vi "CreatePathWriteTrajCSVFile_Example.vi"(11 "Max Velocity M/S":dbl=3.2 format="%17.3f") -> (1 "PathPlannerTrajectory":T2 {"States"."TargetHolonomicRotation"."SIN" format="%13.4f"; "States"."TargetHolonomicRotation"."COS" format="%13.4f"; "States"."TargetHolonomicRotation"."VALUE" format="%13.4f"; "States"."Heading"."SIN" format="%13.4f"; "States"."Heading"."COS" format="%13.4f"; "States"."Heading"."VALUE" format="%13.4f"; "States"."PositionMeters"."Y" format="%14.3f"; "States"."PositionMeters"."X" format="%14.3f"}, 2 "Trajectory State\nCount":i32, 3 "TotalTImeSecs":dbl)   [LabVIEW 2019]
uses:
  <vilib>/Rock Robotics/WPI/ThirdParty/JAS_Junk/TrajLib/Trajectory_Library.lvlib
  <vilib>/Rock Robotics/WPI/ThirdParty/MJansen/PathPlanner/PathPlanner24.lvlib
  <vilib>/Rock Robotics/WPI/ThirdParty/JAS_Junk/TrajLib/TypeDef/TRANSLATION2D.ctl
  <vilib>/Rock Robotics/WPI/ThirdParty/JAS_Junk/TrajLib/TypeDef/ROTATION2D.ctl
  <vilib>/Rock Robotics/WPI/ThirdParty/MJansen/PathPlanner/TypeDef/PathPlannerPathConstraints.ctl
  <vilib>/Rock Robotics/WPI/ThirdParty/MJansen/PathPlanner/TypeDef/PathPlannerTrajectoryState.ctl
  <vilib>/Rock Robotics/WPI/ThirdParty/MJansen/PathPlanner/TypeDef/PathPlannerTrajectory.ctl
panel:
  in  "Trajectory CSV File Name":path=path "sample.csv"
  in  "Optional Comment":string="Sample PathPlanner Trajectory"
  in  "Write File":bool
  out "Trajectory\nWrite error":errorcluster
  in  "End Angle Degrees":dbl format="%#_13g"
  in  "End Velocity M/S":dbl format="%#_13g"
  in  "Start Angual Vel Rad/S":dbl format="%#_13g"
  in  "Start Y Vel M/S":dbl format="%#_13g"
  in  "Start X Vel M/S":dbl format="%#_13g"
  in  "MaxAngularAccel Radians.Sec^2":dbl=2.4 format="%17.3f"
  in  "Point 4":T1={"X Meters"=3.0, "Y Meters"=3.0, "Heading  Deg"=90.0} {"Heading  Deg" format="%13.3f"; "Y Meters" format="%13.3f"; "X Meters" format="%13.3f"}
  in  "Point 3":T1={"X Meters"=3.0, "Y Meters"=2.7, "Heading  Deg"=90.0} {"Heading  Deg" format="%13.3f"; "Y Meters" format="%13.3f"; "X Meters" format="%13.3f"}
  in  "Point 2":T1={"X Meters"=1.3, "Y Meters"=1.0, "Heading  Deg"=0.0} {"Heading  Deg" format="%13.3f"; "Y Meters" format="%13.3f"; "X Meters" format="%13.3f"}
  out "Path\nCreation\nError":bool
  out "Trajectory":cluster{dbl[], dbl[]}(graph)
  in  "Initial Point":T1={"X Meters"=1.0, "Y Meters"=1.0, "Heading  Deg"=0.0} {"Heading  Deg" format="%13.3f"; "Y Meters" format="%13.3f"; "X Meters" format="%13.3f"}
  in  "MaxAcceleration M/S^2":dbl=2.8 format="%17.1f"
  in  "MaxAngularVel  Radians/Sec":dbl=1.8 format="%17.3f"
  # "Create PathPlanner Path/Trajectory Sample"
  # "This VI is designed to be called by BEGIN.VI, but can be executed directly to test trajectory parameters."
  # "CREATED TRAJECTORY INFORMATION"
  # "PATH CONFIGURATION"
  # "PATH DEFINITION"
  # "WRITE TRAJECTORY TO FILE"
  # "There can be as many points as needed."
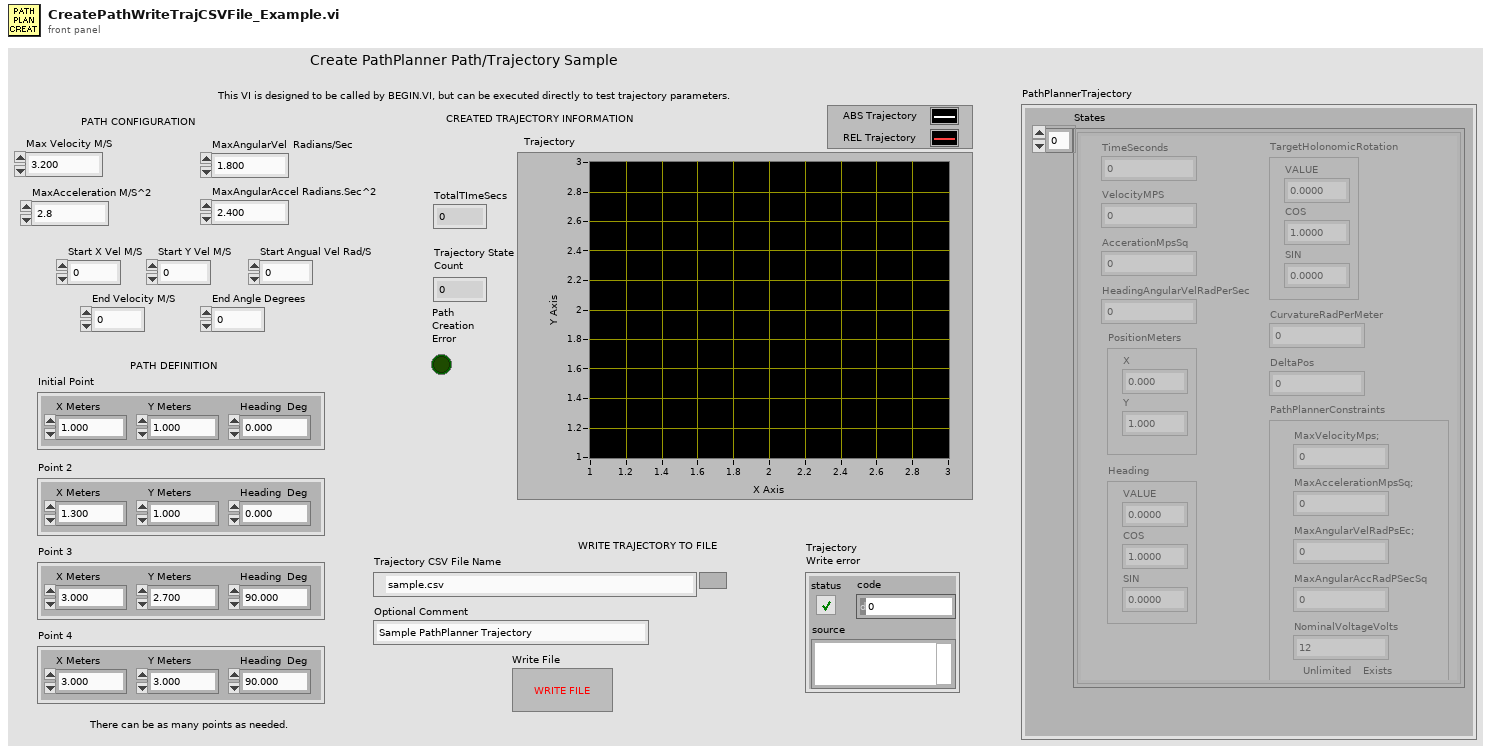
[diagram p1: front panel]
types:
  T1 = cluster{"X Meters":dbl, "Y Meters":dbl, "Heading  Deg":dbl}
  T2 = typedef "PathPlanner24.lvlib/PathPlannerTrajectory.ctl" = cluster{"States":T3[]}
  T3 = typedef "PathPlanner24.lvlib/PathPlannerTrajectoryState.ctl" = cluster{"TimeSeconds":dbl, "VelocityMPS":dbl, "AccerationMpsSq":dbl, "HeadingAngularVelRadPerSec":dbl, "PositionMeters":T4, "Heading":T5, "TargetHolonomicRotation":T5, "CurvatureRadPerMeter":dbl, "PathPlannerConstraints":T6, "DeltaPos":dbl}
  T4 = typedef "Trajectory_Library.lvlib/TRANSLATION2D.ctl" = cluster{"X":dbl, "Y":dbl}
  T5 = typedef "Trajectory_Library.lvlib/ROTATION2D.ctl" = cluster{"VALUE":dbl, "COS":dbl, "SIN":dbl}
  T6 = typedef "PathPlanner24.lvlib/PathPlannerPathConstraints.ctl" = cluster{"MaxVelocityMps;":dbl, "MaxAccelerationMpsSq;":dbl, "MaxAngularVelRadPsEc;":dbl, "MaxAngularAccRadPSecSq":dbl, "Exists":bool, "Unlimited":bool, "NominalVoltageVolts":dbl}
  T7 = typedef "Trajectory_Library.lvlib/POSE2D.ctl" = cluster{"TRANSLATION":T4, "ROTATION":T5}
  T8 = typedef "Trajectory_Library.lvlib/CHASSIS_SPEEDS.ctl" = cluster{"vX":dbl, "vY":dbl, "vOmega":dbl}
  T9 = typedef "PathPlanner24.lvlib/PathPlannerGoalEndState.ctl" = cluster{"VelocityMPS":dbl, "Rotation":T5}
  T10 = typedef "PathPlanner24.lvlib/PathPlannerWaypoint.ctl" = cluster{"prevControl":T4, "anchor":T4, "nextControl":T4, "PrevExists":bool, "NextExists":bool}
  T11 = typedef "PathPlanner24.lvlib/PathPlannerPath.ctl" = cluster{"Reversed":bool, "RotationTargets":T12[], "ConstraintZones":T13[], "EventMarkers":T14[], "GlobalConstraints":T6, "GoalEndState":T9, "AllPoints":T17[], "Name":string, "Waypoints":T10[], "PointTowardsZones":T18[], "IdealStartingState":T19, "IsChoreoPath":bool, "PreventFlipping":bool}
  T12 = typedef "PathPlanner24.lvlib/PathPlannerRotationTarget.ctl" = cluster{"position":dbl, "rotation":T5, "Exists":bool}
  T13 = typedef "PathPlanner24.lvlib/PathPlannerConstraintsZone.ctl" = cluster{"minPosition":dbl, "maxPosition":dbl, "Constraints":T6, "Present":bool}
  T14 = typedef "PathPlanner24.lvlib/PathPlannerEventMarker.ctl" = cluster{"Position":dbl, "Command":T15, "TriggerName":string, "EndPosition":dbl}
  T15 = typedef "PathPlanner24.lvlib/PathPlannerCommandUtil.ctl" = cluster{"waitTime":dbl, "name":string, "pathName":string, "commands":cluster{"type":T16, "waitTime":dbl, "name":string, "pathName":string}[], "type":T16}
  T16 = typedef "PathPlanner24.lvlib/PathPlanner_CommandUtilType_ENUM.ctl" = enum16{"Unknown", "Wait", "Named", "Path", "Sequential", "Parallel", "Race", "Deadline"}
  T17 = typedef "PathPlanner24.lvlib/PathPlannerPathPoint.ctl" = cluster{"Position":T4, "DistAlongPath":dbl, "MaxV":dbl, "Constraints":T6, "RotationTarget":T12, "WaypointRelativePos":dbl}
  T18 = typedef "PathPlanner24.lvlib/PathPlannerPointTowardsZone.ctl" = cluster{"RotationOffset":T5, "Name":string, "TargetPosition":T4, "MinPosition":dbl, "MaxPosition":dbl}
  T19 = typedef "PathPlanner24.lvlib/PathPlannerIdealStartingState.ctl" = cluster{"VelocityMPS":dbl, "Rotation":T5}
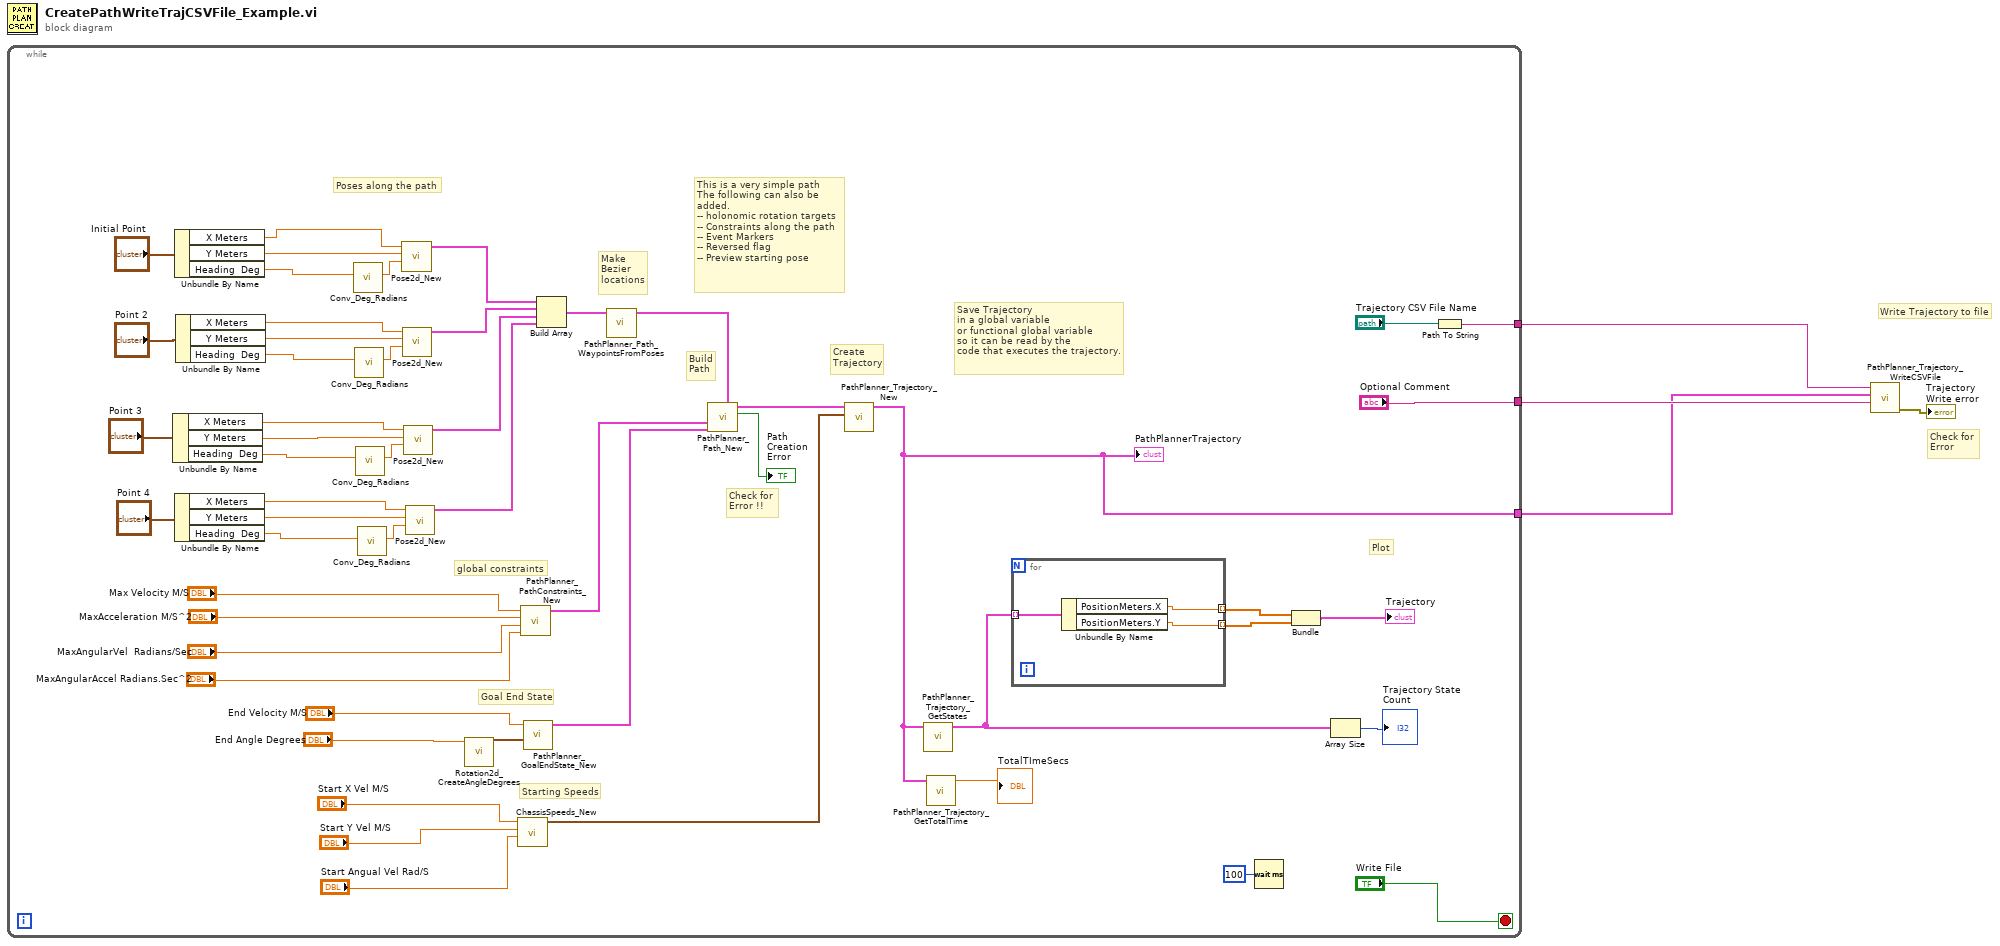
[diagram p0: block diagram]
diagram:
  # "Write Trajectory to file"
  # "Check for\nError"
  n1 = while {
    tunnel: ["Optional Comment"] -> w3
    tunnel: [w8] -> w2
    tunnel: [w7] -> w1
    stop <- "Write File" stop-if-true
    # "This is a very simple path\nThe following can also be\nadded.\n-- holonomic rotation targets\n-- Constraints along the path\n-- Event Markers\n-- Reversed flag\n-- Preview starting pose"
    # "Plot"
    # "Save Trajectory\nin a global variable\nor functional global variable\nso it can be read by the \ncode that executes the trajectory."
    # "Create\nTrajectory"
    # "Check for\nError !!"
    # "Starting Speeds"
    # "Goal End State"
    # "global constraints"
    # "Make\nBezier\nlocations"
    # "Build\nPath"
    # "Poses along the path"
    n2 = Unbundle By Name("Point 3") -> ("X Meters"=w21:dbl, "Y Meters"=w20:dbl, "Heading  Deg"=w19:dbl)
    n3 = Unbundle By Name("Initial Point") -> ("X Meters"=w29:dbl, "Y Meters"=w28:dbl, "Heading  Deg"=w27:dbl)
    n4 = Unbundle By Name("Point 4") -> ("X Meters"=w18:dbl, "Y Meters"=w17:dbl, "Heading  Deg"=w16:dbl)
    n5 = Unbundle By Name("Point 2") -> ("X Meters"=w26:dbl, "Y Meters"=w25:dbl, "Heading  Deg"=w24:dbl)
    n6 = call <vilib>:"Conv_Deg_Radians.vi"("Degress"=w27) -> ("Radians"=w38:dbl)  [unwired: 10 in]
    n7 = call <vilib>:"Conv_Deg_Radians.vi"("Degress"=w24) -> ("Radians"=w39:dbl)  [unwired: 10 in]
    n8 = call <vilib>:"Conv_Deg_Radians.vi"("Degress"=w19) -> ("Radians"=w40:dbl)  [unwired: 10 in]
    n9 = call <vilib>:"Conv_Deg_Radians.vi"("Degress"=w16) -> ("Radians"=w41:dbl)  [unwired: 10 in]
    n10 = call <vilib>:"Pose2d_New.vi"("Heading"=w38, "Y"=w28, "X"=w29) -> ("out POSe"=w42:T7)  [unwired: 8 in]
    n11 = call <vilib>:"Pose2d_New.vi"("Heading"=w39, "Y"=w25, "X"=w26) -> ("out POSe"=w43:T7)  [unwired: 8 in]
    n12 = call <vilib>:"Pose2d_New.vi"("Heading"=w40, "Y"=w20, "X"=w21) -> ("out POSe"=w44:T7)  [unwired: 8 in]
    n13 = call <vilib>:"Pose2d_New.vi"("Heading"=w41, "Y"=w17, "X"=w18) -> ("out POSe"=w45:T7)  [unwired: 8 in]
    n14 = call <vilib>:"Rotation2d_CreateAngleDegrees.vi"("Angle_Degrees"="End Angle Degrees") -> ("ROTATION"=w49:T5)  [unwired: 10 in]
    n15 = call <vilib>:"ChassisSpeeds_New.vi"("vAngular"="Start Angual Vel Rad/S", "vY"="Start Y Vel M/S", "vX"="Start X Vel M/S") -> ("CHASSIS"=w56:T8)  [unwired: 8 in]
    n16 = call <vilib>:"PathPlanner_PathConstraints_New.vi"("MaxAngularAccRadPSecSq"="MaxAngularAccel Radians.Sec^2", "MaxAngularVelRadPsEc;"="MaxAngularVel  Radians/Sec", "MaxAccelerationMpsSq;"="MaxAcceleration M/S^2", "MaxVelocityMps;"="Max Velocity M/S") -> ("PathPlannerConstraints"=w47:T6)  [unwired: 7 in]
    n17 = call <vilib>:"PathPlanner_GoalEndState_New.vi"("Rotation"=w49, "VelocityMPS"="End Velocity M/S") -> ("GoalEndState"=w51:T9)  [unwired: 9 in]
    n18 = Build Array(w42, w43, w44, w45) -> (w37:T7[])
    n19 = call <vilib>:"PathPlanner_Path_WaypointsFromPoses.vi"("Poses"=w37) -> ("Waypoints"=w46:T10[])  [unwired: 9 in, 1 out]
    n20 = call <vilib>:"PathPlanner_Path_New.vi"("Waypoints"=w46, "GoalEndState"=w51, "GlobalConstraints"=w47) -> ("Error"=→"Path\nCreation\nError":bool, "PathPlannerPath"=w52:T11)  [unwired: 7 in]
    n21 = call <vilib>:"PathPlanner_Trajectory_New.vi"("StartingSpeeds"=w56, "Path"=w52) -> ("PathPlannerTrajectory"=w7:T2)  [unwired: 8 in, 1 out]
    "PathPlannerTrajectory" <- w7
    n22 = call <vilib>:"PathPlanner_Trajectory_GetStates.vi"("PathPlannerTrajectory"=w7) -> ("PathPlannerStates"=w33:T3[])  [unwired: 10 in]
    n23 = call <vilib>:"PathPlanner_Trajectory_GetTotalTime.vi"("PathPlannerTrajectory"=w7) -> ("TotalTimeSeconds"=→"TotalTImeSecs":dbl)  [unwired: 10 in]
    n24 = for {
      tunnel: [w60] -> w35 mode=indexing
      tunnel: [w59] -> w36 mode=indexing
      tunnel: w33 -> [w58] mode=indexing
      n25 = Unbundle By Name(w58) -> ("PositionMeters.X"=w60:dbl, "PositionMeters.Y"=w59:dbl)
    }
    n26 = Wait (ms)(milliseconds to wait=u32 100) -> ()  [unwired: 1 out]
    n27 = Bundle(w35, w36) -> (→"Trajectory":cluster{dbl[], dbl[]})  [unwired: 1 in]
    n28 = Array Size(array=w33) -> (size(s)=→"Trajectory State\nCount":i32)
    n29 = Path To String(path="Trajectory CSV File Name") -> (string=w8:string)
  }
  n30 = call <vilib>:"PathPlanner_Trajectory_WriteCSVFile.vi"("Comment"=w3, "TRAJECTORY"=w1, "FileName"=w2) -> ("error out"=→"Trajectory\nWrite error":errorcluster)  [unwired: 8 in]
